vi "VITree.vi"   [LabVIEW 2016, in "DronaTest.lvlib"]
uses:
  DronaTest.lvlib
  APIs/Stimulus/ControlValue/typedef/Name&Occurrence.ctl
  APIs/Assert/AssertControlValue/AlmostEqual.vi
  APIs/Assert/AssertControlValue/Equal.vi
  APIs/Assert/AssertControlValue/NotEqual.vi
  APIs/Assert/AssertControlValue/Greater.vi
  APIs/Assert/AssertControlValue/GreaterOrEqual.vi
  APIs/Assert/AssertControlValue/Less.vi
  APIs/Assert/AssertControlValue/LessOrEqual.vi
  APIs/Assert/AssertControlValue/True.vi
  APIs/Assert/AssertControlValue/False.vi
  APIs/Assert/AssertControlProperty/AssertControlDisable/AssertDisabled.vi
  APIs/Assert/AssertControlProperty/AssertControlDisable/AssertDisabledAndGrayedOut.vi
  APIs/Assert/AssertControlProperty/AssertControlDisable/AssertEnabled.vi
  APIs/Assert/AssertControlValue/Controls/Listbox/AssertValueByFocusIndex.vi
  APIs/Assert/AssertControlValue/Controls/Listbox/AssertValueByFocusName.vi
  APIs/Assert/AssertControlValue/Controls/Listbox/AssertValueByArrayIndex.vi
  APIs/Assert/AssertControlValue/Controls/Listbox/AssertValueByArrayName.vi
  APIs/Assert/AssertControlValue/Controls/Listbox/AssertIndexValue.vi
  APIs/Assert/AssertControlValue/Controls/Listbox/AssertAllItems.vi
  APIs/Assert/AssertControlValue/Controls/Listbox/AssertDisabledItems.vi
  APIs/Assert/AssertControlValue/Controls/MC Listbox/AssertValueByFocusIndex.vi
  APIs/Assert/AssertControlValue/Controls/MC Listbox/AssertValueByFocusName.vi
  APIs/Assert/AssertControlValue/Controls/MC Listbox/AssertValueByArrayIndex.vi
  APIs/Assert/AssertControlValue/Controls/MC Listbox/AssertValueByArrayName.vi
  APIs/Assert/AssertControlValue/Controls/MC Listbox/AssertIndexValue.vi
  APIs/Assert/AssertControlValue/Controls/MC Listbox/AssertAllItems.vi
  APIs/Assert/AssertControlValue/Controls/MC Listbox/AssertDisabledItems.vi
  APIs/Assert/AssertControlValue/Controls/Subpanel/AssertSubpanelVIExecBad.vi
  APIs/Assert/AssertControlValue/Controls/Subpanel/AssertSubpanelVIExecIdle.vi
  APIs/Assert/AssertControlValue/Controls/Subpanel/AssertSubpanelVIExecNotBad.vi
  APIs/Assert/AssertControlValue/Controls/Subpanel/AssertSubpanelVIExecRunning.vi
  APIs/Assert/AssertControlValue/Controls/Subpanel/AssertSubpanelVI.vi
  APIs/Assert/AssertVI/Exec/AssertVIExecBad.vi
  APIs/Assert/AssertVI/Exec/AssertVIExecIdle.vi
  APIs/Assert/AssertVI/Exec/AssertVIExecNotBad.vi
  APIs/Assert/AssertVI/Exec/AssertVIExecRunning.vi
  APIs/Assert/AssertControlProperty/AssertControlVisible/AssertVisible.vi
  APIs/Assert/AssertControlProperty/AssertControlVisible/AssertInvisible.vi
  APIs/Assert/AssertControlValue/Controls/Table/AssertCellValue.vi
  APIs/Assert/AssertControlValue/Controls/Table/AssertRowValue.vi
  APIs/Assert/AssertControlValue/Controls/Table/AssertColumnValue.vi
  APIs/Assert/AssertControlValue/Controls/Table/AssertAllItems.vi
  APIs/Assert/AssertControlValue/Controls/Tree/AssertValueByFocusTag.vi
  APIs/Assert/AssertControlValue/Controls/Tree/AssertValueByFocusNamePath.vi
  APIs/Assert/AssertControlValue/Controls/Tree/AssertValueByArrayTags.vi
  APIs/Assert/AssertControlValue/Controls/Tree/AssertValueByArrayPath.vi
  APIs/Assert/AssertControlValue/Controls/Tree/AssertAllTags.vi
  APIs/Assert/AssertVI/FPState/AssertVIFPStateInvalid.vi
  APIs/Assert/AssertVI/FPState/AssertVIFPStateStandard.vi
  APIs/Assert/AssertVI/FPState/AssertVIFPStateClosed.vi
  APIs/Assert/AssertVI/FPState/AssertVIFPStateHidden.vi
  APIs/Assert/AssertVI/FPState/AssertVIFPStateMinimized.vi
  APIs/Assert/AssertVI/FPState/AssertVIFPStateMaximized.vi
  APIs/Get/GetControlValue/GetControlValueByPathString.vi
  APIs/Get/GetControlRef/GetControlRefByPath.vi
  APIs/Get/GetVI/GetVIByName.vi
  APIs/Get/GetVI/GetVIByPath.vi
  APIs/Stimulus/VI/RunVI.vi
  APIs/Stimulus/VI/OpenVIFrontPanel.vi
  APIs/Stimulus/VI/MakeVIFrontMost.vi
  APIs/Stimulus/VI/CloseVI.vi
  APIs/Stimulus/ControlValue/SetValueAuto.vi
  APIs/Stimulus/ControlValue/ValueSignalByPathString.vi
  APIs/Stimulus/ControlValue/ValueSignalLatchBooleanString.vi
  APIs/Stimulus/ControlValue/Controls/Listbox/SetValueByItemIndex.vi
  APIs/Stimulus/ControlValue/Controls/Listbox/SetValueByItemName.vi
  APIs/Stimulus/ControlValue/Controls/Listbox/SetValueByArrayIndex.vi
  APIs/Stimulus/ControlValue/Controls/Listbox/SetValueByArrayName.vi
  APIs/Stimulus/ControlValue/Controls/MC Listbox/SetValueByItemIndex.vi
  APIs/Stimulus/ControlValue/Controls/MC Listbox/SetValueByItemName.vi
  APIs/Stimulus/ControlValue/Controls/MC Listbox/SetValueByArrayIndex.vi
  APIs/Stimulus/ControlValue/Controls/MC Listbox/SetValueByArrayName.vi
  APIs/Stimulus/ControlValue/Controls/Table/EditCellValue.vi
  APIs/Stimulus/ControlValue/Controls/Table/EditRowValue.vi
  APIs/Stimulus/ControlValue/Controls/Table/EditColumnValue.vi
  APIs/Stimulus/ControlValue/Controls/Table/SetValue.vi
  APIs/Stimulus/ControlValue/Controls/Tree/SetValueByItemTag.vi
  APIs/Stimulus/ControlValue/Controls/Tree/SetValueByHierarchicalPath.vi
  APIs/Stimulus/ControlValue/Controls/Tree/SetValueByItemTagArray.vi
  APIs/Stimulus/ControlValue/Controls/Tree/SetValueByHierarchicalPathArray.vi
  Drona.lvlib
  APIs/Get/GetVI/GetVI.lvlib
  APIs/Get/GetControlValue/GetControlValue.lvlib
  APIs/Get/GetControlRef/GetControlRef.lvlib
  APIs/Stimulus/ControlValue/ControlValue.lvlib
  APIs/Stimulus/ControlValue/Controls/Listbox/StimulusListbox.lvlib
  APIs/Stimulus/ControlValue/Controls/MC Listbox/StimulusMCListbox.lvlib
  APIs/Stimulus/ControlValue/Controls/Table/StimulusTable.lvlib
  APIs/Stimulus/ControlValue/Controls/Tree/StimulusTree.lvlib
  APIs/Assert/AssertControlValue/AssertControlValue.lvlib
  APIs/Assert/AssertControlValue/Controls/MC Listbox/AssertMCListbox.lvlib
  APIs/Assert/AssertControlValue/Controls/Listbox/AssertListbox.lvlib
  APIs/Stimulus/VI/VI.lvlib
  APIs/Assert/AssertControlValue/Controls/Table/AssertTable.lvlib
  APIs/Assert/AssertControlValue/Controls/Tree/AssertTree.lvlib
  APIs/Assert/AssertControlValue/Controls/Subpanel/AssertSubpanel.lvlib
  APIs/Assert/AssertVI/AssertVI.lvlib
  APIs/Assert/AssertControlProperty/AssertControlDisable/AssertControlDisable.lvlib
  APIs/Assert/AssertControlProperty/AssertControlVisible/AssertControlVisible.lvlib
types:
  T1 = typedef "Drona.lvlib/ControlValue.lvlib/Name&Occurrence.ctl" = cluster{"ItemName":string, "Occurrence":i32}
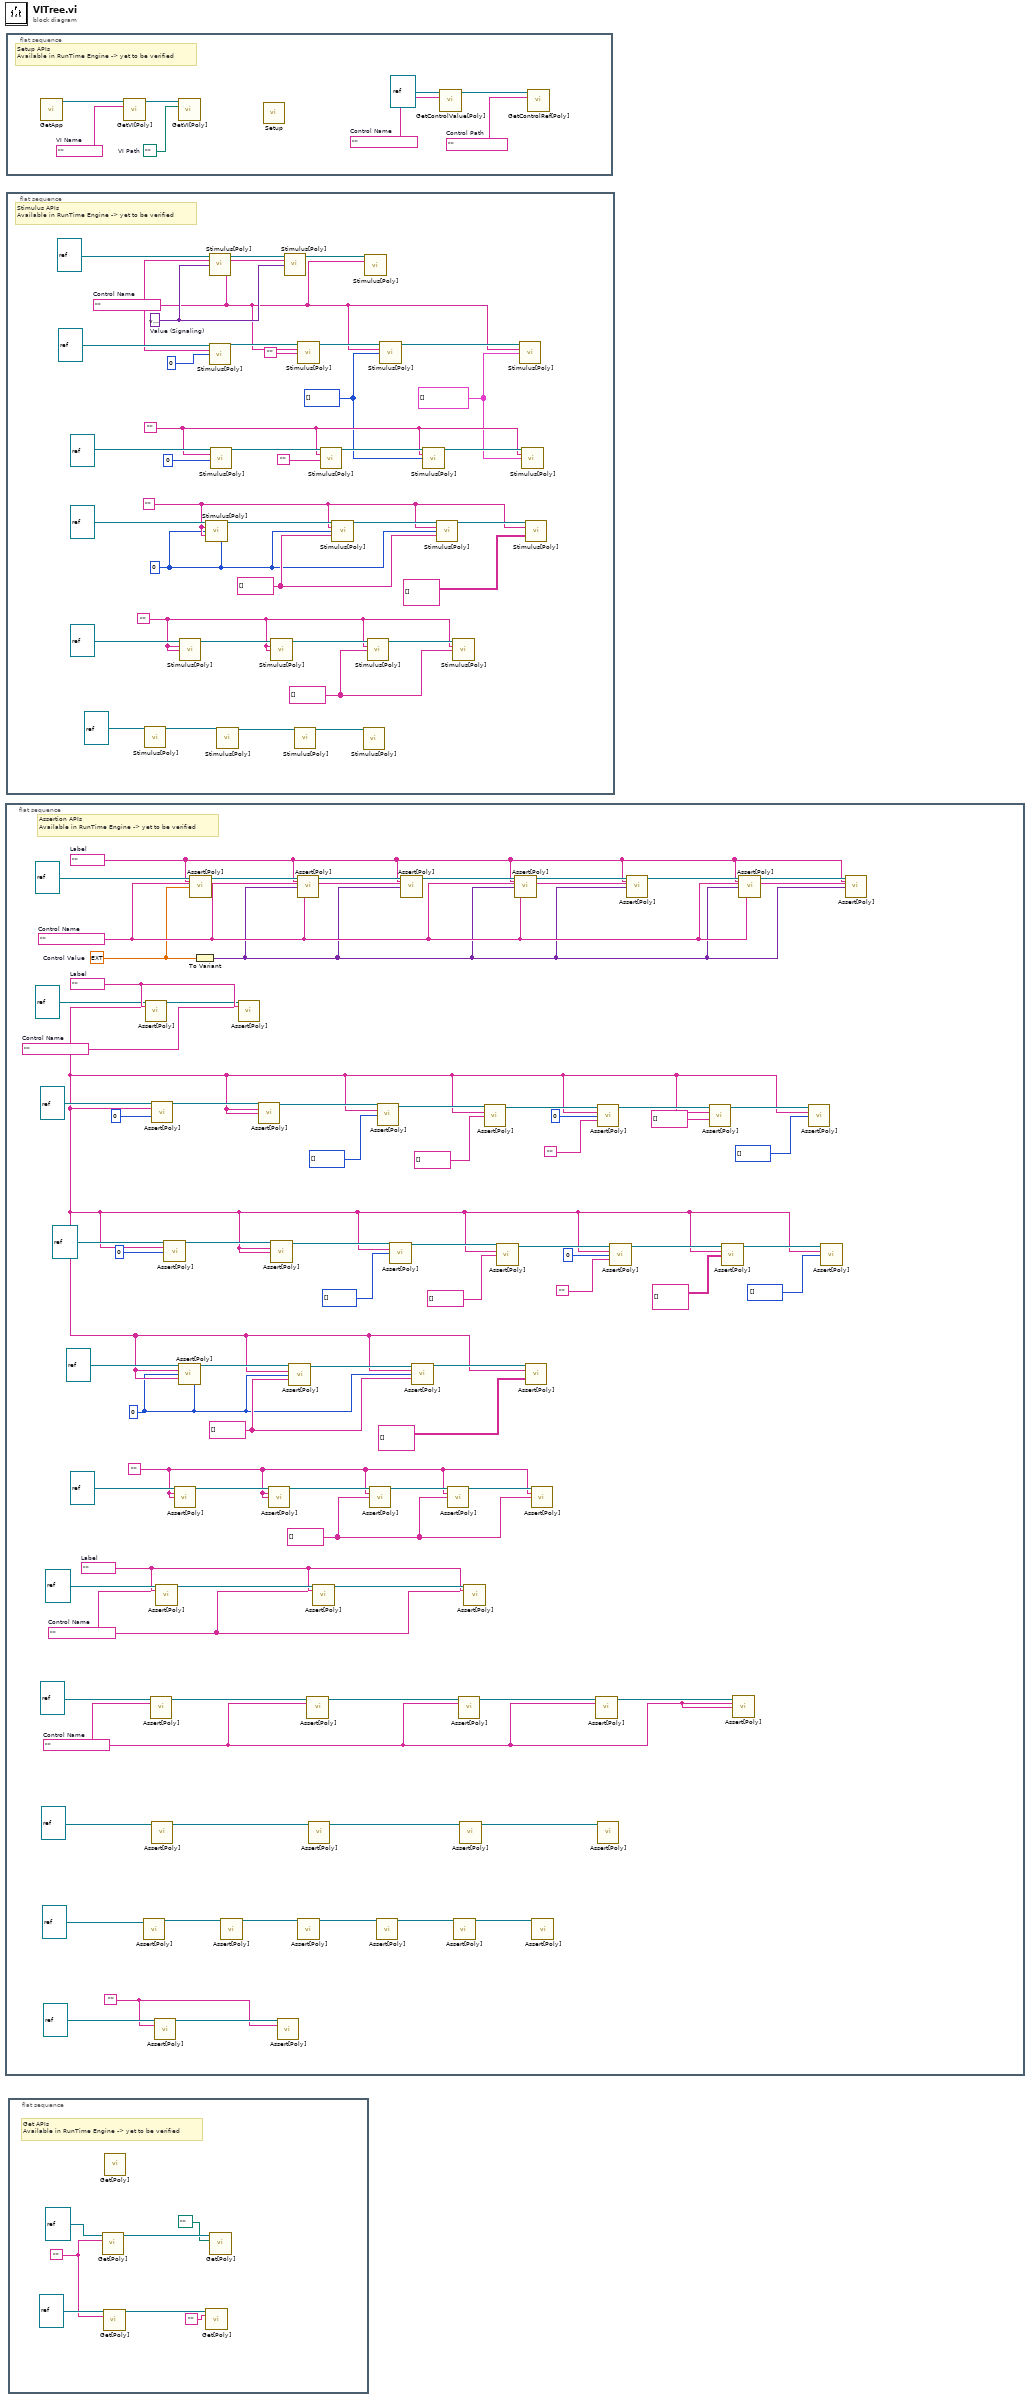
[diagram p0: block diagram]
diagram:
  n1 = flat-sequence {
    frame #0 {
      w9 = string[] [] ("Focus Item Tag")
      w10 = "" ("Control Path")
      w17 = string[] [] ("Item Value")
      w16 = 0 ("Row Index")
      w23 = "" ("Control Path")
      w30 = ""  # Control Name
      w64 = ""  # Control Name
      w65 = ""  # Label
      w18 = ""  # Control Name
      w71 = ""  # Label
      w72 = ext 0.0  # Control Value
      w73 = ""  # Control Name
      w74 = ""  # Label
      # "Assertion APIs\nAvailable in RunTime Engine -> yet to be verified"
      n2 = call-poly "Assert[Poly].vi"("VI Reference In"=refnum<vi> refnum) -> ("VI Reference Out"=w7:refnum<vi>)  [unwired: 12 in, 2 out]
      n3 = call-poly "Assert[Poly].vi"("VI Reference In"=refnum<vi> refnum, "Test Label"=w71, "Control Path"=w18) -> ("VI Reference Out"=w70:refnum<vi>)  [unwired: 10 in, 2 out]
      n4 = call-poly "Assert[Poly].vi"("VI Reference In"=refnum<vi> refnum, "Control Path"=w30) -> ("VI Reference Out"=w34:refnum<vi>)  [unwired: 11 in, 2 out]
      n5 = call-poly "Assert[Poly].vi"("VI Reference In"=refnum<vi> refnum, "Control Path"=w18, "Focus Index"=0) -> ("VI Reference Out"=w62:refnum<vi>)  [unwired: 10 in, 2 out]
      n6 = call-poly "Assert[Poly].vi"("VI Reference In"=refnum<vi> refnum) -> ("VI Reference Out"=w28:refnum<vi>)  [unwired: 12 in, 2 out]
      n7 = call-poly "Assert[Poly].vi"("VI Reference In"=refnum<vi> refnum, "Control Path"=w23) -> ("VI Reference Out"=w25:refnum<vi>)  [unwired: 11 in, 2 out]
      n8 = call-poly "Assert[Poly].vi"("VI Reference In"=refnum<vi> refnum, "Test Label"=w65, "Control Path"=w64) -> ("VI Reference Out"=w67:refnum<vi>)  [unwired: 10 in, 2 out]
      n9 = call-poly "Assert[Poly].vi"("VI Reference In"=refnum<vi> refnum, "Control Path"=w18, "Focus Index"=0) -> ("VI Reference Out"=w48:refnum<vi>)  [unwired: 10 in, 2 out]
      n10 = call-poly "Assert[Poly].vi"("VI Reference In"=refnum<vi> refnum, "Control Path"=w10, "Focus Item Tag"=w10) -> ("VI Reference Out"=w14:refnum<vi>)  [unwired: 10 in, 2 out]
      n11 = call-poly "Assert[Poly].vi"("VI Reference In"=refnum<vi> refnum, "Control Path"=w18, "Row Index"=w16, "Item Value"=w18, "Column Index"=w16) -> ("VI Reference Out"=w21:refnum<vi>)  [unwired: 8 in, 2 out]
      n12 = call-poly "Assert[Poly].vi"("VI Reference In"=refnum<vi> refnum, "Test Label"=w74, "Control Path"=w73, "Control Value"=w72) -> ("VI Reference Out"=w80:refnum<vi>)  [unwired: 9 in, 2 out]
      n13 = To Variant(anything=w72) -> (Variant=w2:variant)
      n14 = call-poly "Assert[Poly].vi"("VI Reference In"=w7) -> ("VI Reference Out"=w6:refnum<vi>)  [unwired: 12 in, 2 out]
      n15 = call-poly "Assert[Poly].vi"("VI Reference In"=w70, "Test Label"=w71, "Control Path"=w18) -> ()  [unwired: 10 in, 3 out]
      n16 = call-poly "Assert[Poly].vi"("VI Reference In"=w62, "Control Path"=w18, "Item Name"=w18) -> ("VI Reference Out"=w61:refnum<vi>)  [unwired: 10 in, 2 out]
      n17 = call-poly "Assert[Poly].vi"("VI Reference In"=w14, "Control Path"=w10, "Focus Item Path"=w10) -> ("VI Reference Out"=w13:refnum<vi>)  [unwired: 10 in, 2 out]
      n18 = call-poly "Assert[Poly].vi"("VI Reference In"=w48, "Control Path"=w18, "Item Name"=w18) -> ("VI Reference Out"=w47:refnum<vi>)  [unwired: 10 in, 2 out]
      n19 = call-poly "Assert[Poly].vi"("VI Reference In"=w25, "Control Path"=w23) -> ()  [unwired: 11 in, 3 out]
      n20 = call-poly "Assert[Poly].vi"("VI Reference In"=w21, "Control Path"=w18, "Row Index"=w16, "Item Value"=w17) -> ("VI Reference Out"=w20:refnum<vi>)  [unwired: 9 in, 2 out]
      n21 = call-poly "Assert[Poly].vi"("VI Reference In"=w80, "Test Label"=w74, "Control Path"=w73, "Control Value"=w2) -> ("VI Reference Out"=w79:refnum<vi>)  [unwired: 9 in, 2 out]
      n22 = call-poly "Assert[Poly].vi"("VI Reference In"=w6) -> ("VI Reference Out"=w5:refnum<vi>)  [unwired: 12 in, 2 out]
      n23 = call-poly "Assert[Poly].vi"("VI Reference In"=w34, "Control Path"=w30) -> ("VI Reference Out"=w33:refnum<vi>)  [unwired: 11 in, 2 out]
      n24 = call-poly "Assert[Poly].vi"("VI Reference In"=w28) -> ("VI Reference Out"=w27:refnum<vi>)  [unwired: 12 in, 2 out]
      n25 = call-poly "Assert[Poly].vi"("VI Reference In"=w67, "Test Label"=w65, "Control Path"=w64) -> ("VI Reference Out"=w66:refnum<vi>)  [unwired: 10 in, 2 out]
      n26 = call-poly "Assert[Poly].vi"("VI Reference In"=w13, "Control Path"=w10, "Focus Item Tag"=w9) -> ("VI Reference Out"=w12:refnum<vi>)  [unwired: 10 in, 2 out]
      n27 = call-poly "Assert[Poly].vi"("VI Reference In"=w5) -> ("VI Reference Out"=w4:refnum<vi>)  [unwired: 12 in, 2 out]
      n28 = call-poly "Assert[Poly].vi"("VI Reference In"=w61, "Control Path"=w18, "Focus Item Index"=i32[] []) -> ("VI Reference Out"=w60:refnum<vi>)  [unwired: 10 in, 2 out]
      n29 = call-poly "Assert[Poly].vi"("VI Reference In"=w47, "Control Path"=w18, "Focus Item Index"=i32[] []) -> ("VI Reference Out"=w46:refnum<vi>)  [unwired: 10 in, 2 out]
      n30 = call-poly "Assert[Poly].vi"("VI Reference In"=w79, "Test Label"=w74, "Control Path"=w73, "Control Value"=w2) -> ("VI Reference Out"=w78:refnum<vi>)  [unwired: 9 in, 2 out]
      n31 = call-poly "Assert[Poly].vi"("VI Reference In"=w20, "Control Path"=w18, "Column Index"=w16, "Item Value"=w17) -> ("VI Reference Out"=w19:refnum<vi>)  [unwired: 9 in, 2 out]
      n32 = call-poly "Assert[Poly].vi"("VI Reference In"=w12, "Control Path"=w10, "Focus Item Path"=w9) -> ("VI Reference Out"=w11:refnum<vi>)  [unwired: 10 in, 2 out]
      n33 = call-poly "Assert[Poly].vi"("VI Reference In"=w4) -> ("VI Reference Out"=w3:refnum<vi>)  [unwired: 12 in, 2 out]
      n34 = call-poly "Assert[Poly].vi"("VI Reference In"=w33, "Control Path"=w30) -> ("VI Reference Out"=w32:refnum<vi>)  [unwired: 11 in, 2 out]
      n35 = call-poly "Assert[Poly].vi"("VI Reference In"=w27) -> ("VI Reference Out"=w26:refnum<vi>)  [unwired: 12 in, 2 out]
      n36 = call-poly "Assert[Poly].vi"("VI Reference In"=w66, "Test Label"=w65, "Control Path"=w64) -> ()  [unwired: 10 in, 3 out]
      n37 = call-poly "Assert[Poly].vi"("VI Reference In"=w60, "Control Path"=w18, "Focus Item Names"=string[] []) -> ("VI Reference Out"=w59:refnum<vi>)  [unwired: 10 in, 2 out]
      n38 = call-poly "Assert[Poly].vi"("VI Reference In"=w46, "Control Path"=w18, "Focus Item Names"=string[] []) -> ("VI Reference Out"=w45:refnum<vi>)  [unwired: 10 in, 2 out]
      n39 = call-poly "Assert[Poly].vi"("VI Reference In"=w78, "Test Label"=w74, "Control Path"=w73, "Control Value"=w2) -> ("VI Reference Out"=w77:refnum<vi>)  [unwired: 9 in, 2 out]
      n40 = call-poly "Assert[Poly].vi"("VI Reference In"=w19, "Control Path"=w18, "Item Value"=string[][] []) -> ()  [unwired: 10 in, 3 out]
      n41 = call-poly "Assert[Poly].vi"("VI Reference In"=w11, "Control Path"=w10, "Item Tags"=w9) -> ()  [unwired: 10 in, 3 out]
      n42 = call-poly "Assert[Poly].vi"("VI Reference In"=w3) -> ()  [unwired: 12 in, 3 out]
      n43 = call-poly "Assert[Poly].vi"("VI Reference In"=w32, "Control Path"=w30) -> ("VI Reference Out"=w31:refnum<vi>)  [unwired: 11 in, 2 out]
      n44 = call-poly "Assert[Poly].vi"("VI Reference In"=w59, "Control Path"=w18, "Item Index"=0, "Item Value"="") -> ("VI Reference Out"=w58:refnum<vi>)  [unwired: 9 in, 2 out]
      n45 = call-poly "Assert[Poly].vi"("VI Reference In"=w26) -> ()  [unwired: 12 in, 3 out]
      n46 = call-poly "Assert[Poly].vi"("VI Reference In"=w45, "Control Path"=w18, "Row Index"=0 ("Item Index"), "Item Value"="") -> ("VI Reference Out"=w44:refnum<vi>)  [unwired: 9 in, 2 out]
      n47 = call-poly "Assert[Poly].vi"("VI Reference In"=w77, "Test Label"=w74, "Control Path"=w73, "Control Value"=w2) -> ("VI Reference Out"=w76:refnum<vi>)  [unwired: 9 in, 2 out]
      n48 = call-poly "Assert[Poly].vi"("VI Reference In"=w58, "Control Path"=w18, "Item Names"=string[] []) -> ("VI Reference Out"=w57:refnum<vi>)  [unwired: 10 in, 2 out]
      n49 = call-poly "Assert[Poly].vi"("VI Reference In"=w44, "Control Path"=w18, "Item Names"=string[][] []) -> ("VI Reference Out"=w43:refnum<vi>)  [unwired: 10 in, 2 out]
      n50 = call-poly "Assert[Poly].vi"("VI Reference In"=w31, "Control Path"=w30, "VI Name"=w30) -> ()  [unwired: 10 in, 3 out]
      n51 = call-poly "Assert[Poly].vi"("VI Reference In"=w76, "Test Label"=w74, "Control Path"=w73, "Control Value"=w2) -> ("VI Reference Out"=w75:refnum<vi>)  [unwired: 9 in, 2 out]
      n52 = call-poly "Assert[Poly].vi"("VI Reference In"=w57, "Control Path"=w18, "Disabled Items"=i32[] []) -> ()  [unwired: 10 in, 3 out]
      n53 = call-poly "Assert[Poly].vi"("VI Reference In"=w43, "Control Path"=w18, "Disabled Items"=i32[] []) -> ()  [unwired: 10 in, 3 out]
      n54 = call-poly "Assert[Poly].vi"("VI Reference In"=w75, "Test Label"=w74, "Control Path"=w73, "Control Value"=w2) -> ()  [unwired: 9 in, 3 out]
    }
  }
  n55 = flat-sequence {
    frame #0 {
      w82 = ""  # Control Path
      w84 = ""  # Control Name
      w86 = path ""  # VI Path
      w87 = ""  # VI Name
      # "Setup APIs\nAvailable in RunTime Engine -> yet to be verified"
      n56 = call "GetApp.vi"() -> ("Application Ref"=w88:refnum<vi>)  [unwired: 14 in, 1 out]
      n57 = call-poly "GetVI[Poly].vi"("Application Ref in"=w88, "VI Name"=w87) -> ("Application Ref out"=w89:refnum<vi>)  [unwired: 11 in, 2 out]
      n58 = call-poly "GetVI[Poly].vi"("Application Ref in"=w89, "VI Path"=w86) -> ()  [unwired: 11 in, 3 out]
      n59 = call "Setup.vi"() -> ()  [unwired: 13 in, 3 out]
      n60 = call-poly "GetControlValue[Poly].vi"("VI Reference In"=refnum<vi> refnum, "Control Path"=w84) -> ("VI Reference Out"=w83:refnum<vi>)  [unwired: 11 in, 2 out]
      n61 = call-poly "GetControlRef[Poly].vi"("VI Reference In"=w83, "Control Path"=w82) -> ()  [unwired: 11 in, 3 out]
    }
  }
  n62 = flat-sequence {
    frame #0 {
      w91 = string[] [] ("Item Tags Array")
      w92 = "" ("Control Path")
      w98 = string[] [] ("Value")
      w90 = 0 ("Item Index")
      w99 = "" ("Control Path")
      w107 = "" ("Control Path")
      w104 = T1[] [] ("Name Array")
      w105 = i32[] [] ("Index Array")
      w121 = variant  # Value (Signaling)
      w115 = ""  # Control Name
      # "Stimulus APIs\nAvailable in RunTime Engine -> yet to be verified"
      n63 = call-poly "Stimulus[Poly].vi"("VI Reference In"=refnum<vi> refnum) -> ("VI Reference Out"=w126:refnum<vi>)  [unwired: 13 in, 1 out]
      n64 = call-poly "Stimulus[Poly].vi"("VI Reference In"=refnum<vi> refnum, "Control Path"=w92, "Item Tag"=w92) -> ("VI Reference Out"=w95:refnum<vi>)  [unwired: 11 in, 1 out]
      n65 = call-poly "Stimulus[Poly].vi"("VI Reference In"=refnum<vi> refnum, "Control Path"=w99, "Row Index"=w90, "Value"=w99, "Column Index"=w90) -> ("VI Reference Out"=w102:refnum<vi>)  [unwired: 9 in, 1 out]
      n66 = call-poly "Stimulus[Poly].vi"("VI Reference In"=refnum<vi> refnum, "Control Path"=w115, "Value (Signaling)"=w121) -> ("VI Reference Out"=w122:refnum<vi>)  [unwired: 11 in, 1 out]
      n67 = call-poly "Stimulus[Poly].vi"("VI Reference In"=refnum<vi> refnum, "Control Path"=w115, "Item Index"=0) -> ("VI Reference Out"=w118:refnum<vi>)  [unwired: 11 in, 1 out]
      n68 = call-poly "Stimulus[Poly].vi"("VI Reference In"=refnum<vi> refnum, "Control Path"=w107, "Item Index"=0) -> ("VI Reference Out"=w111:refnum<vi>)  [unwired: 11 in, 1 out]
      n69 = call-poly "Stimulus[Poly].vi"("VI Reference In"=w126) -> ("VI Reference Out"=w125:refnum<vi>)  [unwired: 13 in, 1 out]
      n70 = call-poly "Stimulus[Poly].vi"("VI Reference In"=w95, "Control Path"=w92, "Hierarchical Path"=w92) -> ("VI Reference Out"=w94:refnum<vi>)  [unwired: 11 in, 1 out]
      n71 = call-poly "Stimulus[Poly].vi"("VI Reference In"=w122, "Control Path"=w115, "Value (Signaling)"=w121) -> ("VI Reference Out"=w120:refnum<vi>)  [unwired: 11 in, 1 out]
      n72 = call-poly "Stimulus[Poly].vi"("VI Reference In"=w125) -> ("VI Reference Out"=w124:refnum<vi>)  [unwired: 13 in, 1 out]
      n73 = call-poly "Stimulus[Poly].vi"("VI Reference In"=w118, "Control Path"=w115, "Item Name"="") -> ("VI Reference Out"=w117:refnum<vi>)  [unwired: 11 in, 1 out]
      n74 = call-poly "Stimulus[Poly].vi"("VI Reference In"=w111, "Control Path"=w107, "Item Name"="") -> ("VI Reference Out"=w110:refnum<vi>)  [unwired: 11 in, 1 out]
      n75 = call-poly "Stimulus[Poly].vi"("VI Reference In"=w102, "Control Path"=w99, "Row Index"=w90, "Value"=w98) -> ("VI Reference Out"=w101:refnum<vi>)  [unwired: 10 in, 1 out]
      n76 = call-poly "Stimulus[Poly].vi"("VI Reference In"=w124) -> ()  [unwired: 13 in, 2 out]
      n77 = call-poly "Stimulus[Poly].vi"("VI Reference In"=w120, "Control Path"=w115) -> ()  [unwired: 12 in, 2 out]
      n78 = call-poly "Stimulus[Poly].vi"("VI Reference In"=w94, "Control Path"=w92, "Item Tags Array"=w91) -> ("VI Reference Out"=w93:refnum<vi>)  [unwired: 11 in, 1 out]
      n79 = call-poly "Stimulus[Poly].vi"("VI Reference In"=w117, "Control Path"=w115, "Index Array"=w105) -> ("VI Reference Out"=w116:refnum<vi>)  [unwired: 11 in, 1 out]
      n80 = call-poly "Stimulus[Poly].vi"("VI Reference In"=w110, "Control Path"=w107, "Index Array"=w105) -> ("VI Reference Out"=w109:refnum<vi>)  [unwired: 11 in, 1 out]
      n81 = call-poly "Stimulus[Poly].vi"("VI Reference In"=w101, "Control Path"=w99, "Column Index"=w90, "Value"=w98) -> ("VI Reference Out"=w100:refnum<vi>)  [unwired: 10 in, 1 out]
      n82 = call-poly "Stimulus[Poly].vi"("VI Reference In"=w93, "Control Path"=w92, "Hierarchical Path Array"=w91) -> ()  [unwired: 11 in, 2 out]
      n83 = call-poly "Stimulus[Poly].vi"("VI Reference In"=w116, "Control Path"=w115, "Name Array"=w104) -> ()  [unwired: 11 in, 2 out]
      n84 = call-poly "Stimulus[Poly].vi"("VI Reference In"=w109, "Control Path"=w107, "Name Array"=w104) -> ()  [unwired: 11 in, 2 out]
      n85 = call-poly "Stimulus[Poly].vi"("VI Reference In"=w100, "Control Path"=w99, "Value"=string[][] []) -> ()  [unwired: 11 in, 2 out]
    }
  }
  n86 = flat-sequence {
    frame #0 {
      w130 = "" ("VI Name")
      # "Get APIs\nAvailable in RunTime Engine -> yet to be verified"
      n87 = call-poly "Get[Poly].vi"("Application Ref in"=refnum<vi> refnum, "VI Name"=w130) -> ("Application Ref out"=w133:refnum<vi>)  [unwired: 11 in, 2 out]
      n88 = call-poly "Get[Poly].vi"("VI Reference In"=refnum<vi> refnum, "Control Path"=w130) -> ("VI Reference Out"=w129:refnum<vi>)  [unwired: 11 in, 2 out]
      n89 = call-poly "Get[Poly].vi"() -> ()  [unwired: 14 in, 2 out]
      n90 = call-poly "Get[Poly].vi"("VI Reference In"=w129, "Control Path"="") -> ()  [unwired: 11 in, 3 out]
      n91 = call-poly "Get[Poly].vi"("Application Ref in"=w133, "VI Path"=path "") -> ()  [unwired: 11 in, 3 out]
    }
  }
